vi "AlliGator Show-Hide Phasor Indicators.vi"(8 "Error In":errorcluster) -> (0 "Error Out":errorcluster)   [LabVIEW 2021, in "AlliGator Phasor Plot.lvlib"]
uses:
  AlliGator Phasor Plot.lvlib
panel:
  # "see the License on the block diagram (Ctrl+E or Window:Show Block Diagram)"
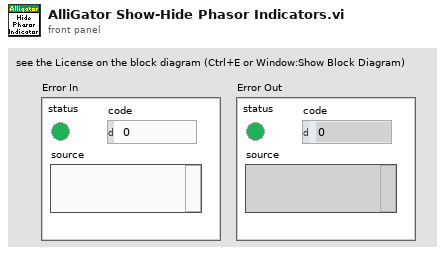
[diagram p1: front panel]
types:
  T1 = typedef "AlliGator Phasor Plot.lvlib/AlliGator Phasor Plot Ctrl Refnums.ctl" = cluster{"Phasor Ratio":refnum<vi>, "Modulus Lifetime":refnum<vi>, "Phasor at cursor (m, phi)":refnum<vi>, "Phase Lifetime":refnum<vi>, "Phasor at cursor (g, s)":refnum<vi>, "Phasor Plor Average Lifetime":refnum<vi>, "Phasor Plot Active":refnum<vi>, "Save Phasor Plot":refnum<vi>, "Image Overlay Color":refnum<vi>, "Phasor Plot Color Scale":refnum<vi>, "Reference 1 Button":refnum<vi>, "Reference 2 Button":refnum<vi>, "True Phasor Plot Value":refnum<vi>, "Phasor Plot Display Range":refnum<vi>, "Phasor Plot Display":refnum<vi>, "Phasor Plot Frequency":refnum<vi>, "Overlay Mode":refnum<vi>}
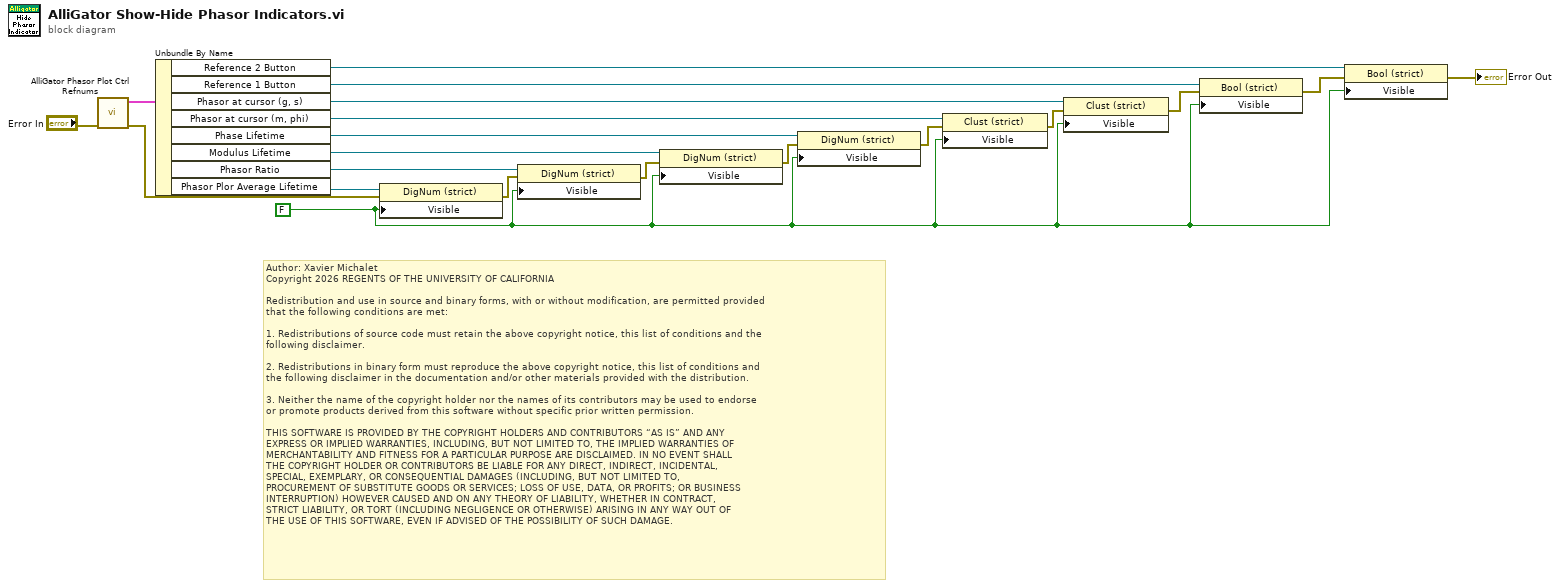
[diagram p0: block diagram]
diagram:
  w2 = FALSE ("Visible")
  # "Author: Xavier Michalet\nCopyright 2026 REGENTS OF THE UNIVERSITY OF CALIFORNIA\n\nRedistribution and use in source and binary forms, with or without modification, are permitted provided\nthat the following conditions are met:\n\n1. Redistributions of source code must retain the above copyright notice, this list of conditions and the\nfollowing disclaimer.\n\n2. Redistributions in binary form must reproduce the above copyright notice, this list of conditions and\nthe following disclaimer in the documentation and/or other materials provided with the distribution.\n\n3. Neither the name of the copyright holder nor the names of its contributors may be used to endorse \nor promote products derived from this software without specific prior written permission.\n\nTHIS SOFTWARE IS PROVIDED BY THE COPYRIGHT HOLDERS AND CONTRIBUTORS “AS IS” AND ANY \nEXPRESS OR IMPLIED WARRANTIES, INCLUDING, BUT NOT LIMITED TO, THE IMPLIED WARRANTIES OF\nMERCHANTABILITY AND FITNESS FOR A PARTICULAR PURPOSE ARE DISCLAIMED. IN NO EVENT SHALL\nTHE COPYRIGHT HOLDER OR CONTRIBUTORS BE LIABLE FOR ANY DIRECT, INDIRECT, INCIDENTAL, \nSPECIAL, EXEMPLARY, OR CONSEQUENTIAL DAMAGES (INCLUDING, BUT NOT LIMITED TO, \nPROCUREMENT OF SUBSTITUTE GOODS OR SERVICES; LOSS OF USE, DATA, OR PROFITS; OR BUSINESS\nINTERRUPTION) HOWEVER CAUSED AND ON ANY THEORY OF LIABILITY, WHETHER IN CONTRACT, \nSTRICT LIABILITY, OR TORT (INCLUDING NEGLIGENCE OR OTHERWISE) ARISING IN ANY WAY OUT OF\nTHE USE OF THIS SOFTWARE, EVEN IF ADVISED OF THE POSSIBILITY OF SUCH DAMAGE."
  n1 = call "AlliGator Phasor Plot Ctrl Refnums.vi"("error in (no error)"="Error In") -> ("error out"=w12:errorcluster, "Phasor Plot Ctrl Refnums"=w18:T1)  [unwired: 9 in]
  n2 = Unbundle By Name(w18) -> ("Reference 2 Button"=w4:refnum<vi>, "Reference 1 Button"=w6:refnum<vi>, "Phasor at cursor (g, s)"=w19:refnum<vi>, "Phasor at cursor (m, phi)"=w20:refnum<vi>, "Phase Lifetime"=w16:refnum<vi>, "Modulus Lifetime"=w15:refnum<vi>, "Phasor Ratio"=w14:refnum<vi>, "Phasor Plor Average Lifetime"=w13:refnum<vi>)
  n3 = property class="DigNum (strict)"(reference=w13, error in=w12, "Visible"=w2) -> (error out=w11:errorcluster)  [unwired: 1 out]
  n4 = property class="DigNum (strict)"(reference=w14, error in=w11, "Visible"=w2) -> (error out=w10:errorcluster)  [unwired: 1 out]
  n5 = property class="DigNum (strict)"(reference=w15, error in=w10, "Visible"=w2) -> (error out=w9:errorcluster)  [unwired: 1 out]
  n6 = property class="DigNum (strict)"(reference=w16, error in=w9, "Visible"=w2) -> (error out=w8:errorcluster)  [unwired: 1 out]
  n7 = property class="Clust (strict)"(reference=w20, error in=w8, "Visible"=w2) -> (error out=w7:errorcluster)  [unwired: 1 out]
  n8 = property class="Clust (strict)"(reference=w19, error in=w7, "Visible"=w2) -> (error out=w5:errorcluster)  [unwired: 1 out]
  n9 = property class="Bool (strict)"(reference=w6, error in=w5, "Visible"=w2) -> (error out=w3:errorcluster)  [unwired: 1 out]
  n10 = property class="Bool (strict)"(reference=w4, error in=w3, "Visible"=w2) -> (error out=→"Error Out":errorcluster)  [unwired: 1 out]
